vi "PSCreatePngTextChunk.vi"(10 "Contents":string, 11 "Keyword":string) -> (3 "PNG Chunk":string)   [LabVIEW 2013, in "VIVendor.lvlib" / "VVPngSnippet.lvlib"]
doc: "Creates a PNG tEXt chunk.\n\nIn the format:\nKeyword /00 Data\n\nCode by Darin\n\nOrigin:\n* PNG Snippet VIs from Code Complete Tool\n* http://sourceforge.net/projects/lv-cct-tool/\n* Commit: 9d97aea5cbd2fc456c5914801e927df6a901d523\n* License: BSD -- see NOTICE.txt"
uses:
  VVPngSnippet.lvlib
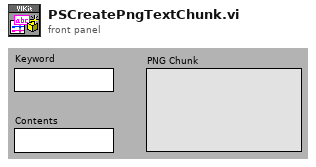
[diagram p1: front panel]
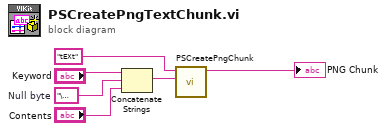
[diagram p0: block diagram]
diagram:
  w3 = "\u0000"  # Null byte
  n1 = Concatenate Strings("Keyword", w3, "Contents") -> (w1:string)
  n2 = call "PSCreatePngChunk.vi"("Data"=w1, "Name"="tEXt") -> ("PNG Chunk"=→"PNG Chunk":string)  [unwired: 9 in]
